vi "Extract_complete_frames.vi"(9 "Frame_leng":i32=1 min=1 step=1, 10 "Frame_head":string, 11 "Source_data":string) -> (3 "Result_ARR_data":string[](array[string]))   [LabVIEW 2025, in "Procotol_class.lvclass"]
uses:
  Procotol_class.lvclass
panel:
  out "Remaining_data":string
  # "包含帧头的奥"
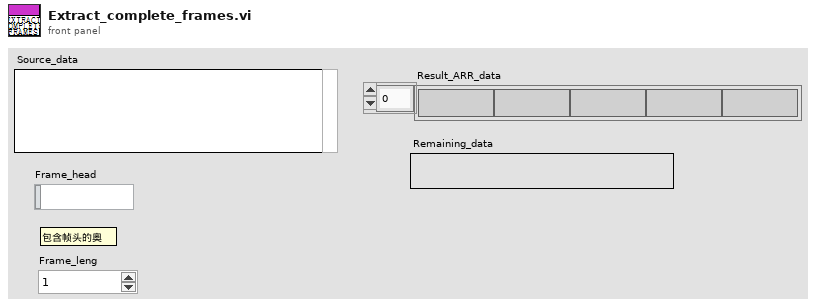
[diagram p1: front panel]
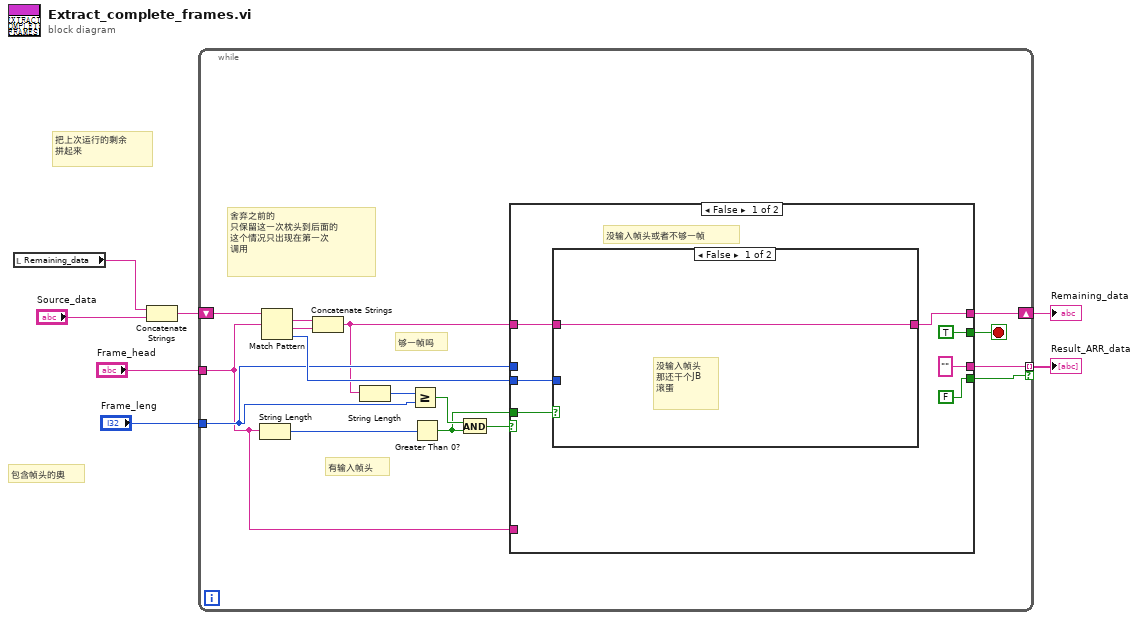
[diagram p0: block diagram]
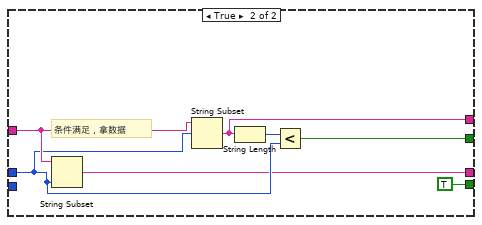
[diagram p3: hidden frame]
diagram:
  # "包含帧头的奥"
  # "把上次运行的剩余\n拼起来"
  n1 = local read "Remaining_data"() -> (w7:string)
  n2 = Concatenate Strings(w7, "Source_data") -> (w5:string)
  n3 = while {
    shift-right: [w17] -> w4
    shift-left: w5 -> [w14]
    tunnel: "Frame_head" -> [w12]
    tunnel: "Frame_leng" -> [w13]
    tunnel: [w10] -> w1 mode=indexing if=w9
    stop <- w16 stop-if-true
    # "有输入帧头"
    # "够一帧吗"
    # "舍弃之前的\n只保留这一次枕头到后面的\n这个情况只出现在第一次\n调用"
    n4 = String Length ("字符串长度")(string=w12) -> (length=w11:i32)
    n5 = Match Pattern ("匹配模式")(string=w14, regular expression=w12) -> (match substring=w23:string, after substring=w22:string, offset past match=w15:i32)  [unwired: 1 in, 1 out]
    n6 = Concatenate Strings(w23, w22) -> (w8:string)
    n7 = String Length ("字符串长度")(string=w8) -> (length=w21:i32)
    n8 = Greater Or Equal?(x=w21, y=w13) -> (x >= y?=w20:bool)
    n9 = Greater Than 0?(x=w11) -> (x > 0?=w18:bool)
    n10 = And(x=w20, y=w18) -> (x .and. y?=w19:bool)
    n11 = case shown="False" w19 {
      tunnel: w18 -> [w30 _]
      tunnel: [w29 w37] -> w17
      tunnel: [TRUE w35] -> w16
      tunnel: w15 -> [w28 _]
      tunnel: w8 -> [w27 w39]
      tunnel: w13 -> [_ w38]
      tunnel: w12 -> [_ _]
      tunnel: ["" w36] -> w10
      tunnel: [FALSE TRUE ("x < y?")] -> w9
      frame False {
        # "没输入帧头或者不够一帧"
        n12 = case shown="False" w30 {
          tunnel: [w31 w32] -> w29
          tunnel: w28 -> [_ _]
          tunnel: w27 -> [w31 w32]
          frame False {
            # "没输入帧头\n那还干个JB\n滚蛋"
          }
          frame True {
            # "长度不够，啥也不干，爱咋咋的"
            # "输入了帧头"
          }
        }
      }
      frame True {
        # "条件满足，拿数据"
        n13 = String Subset ("截取字符串")(string=w39, length (rest)=w38) -> (substring=w36:string)  [unwired: 1 in]
        n14 = String Subset(string=w39, offset (0)=w38) -> (substring=w37:string)  [unwired: 1 in]
        n15 = String Length(string=w37) -> (length=w33:i32)
        n16 = Less?(x=w33, y=w38) -> (x < y?=w35:bool)
      }
    }
  }
  "Remaining_data" <- w4
  "Result_ARR_data" <- w1
